vi "Measurement Logic.vi"(8 "error in":errorcluster, 9 "measurement configuration":T2 {"PAYLOAD" format="%x"; "TYPE" items=["CAN Data"=0, "CAN Remote"=1, "CAN Bus Error"=2, "CAN 2.0 Data"=8, "CAN FD Data"=16, "CAN FD+BRS Data"=24, "J1939 Data"=192, "Delay"=224, "Log Trigger"=225, "Start Trigger"=226]; "IDENTIFIER" format="%x"; "Baudrate" format="%x"; "FD Baudrate" format="%x"}, 10 "measure call context in":refnum<class "Measure Call Context.lvclass">) -> (0 "error out":errorcluster, 1 "measurement results":T1, 2 "measure call context out":refnum<class "Measure Call Context.lvclass">)   [LabVIEW 2025, in "CAN-LIN Frame Generator.lvclass"]
doc: "Contains the core logic for executing the measurement."
uses:
  CAN-LIN Frame Generator.lvclass
  <vilib>/Plug-In SDKs/Measurements/Measure Call Context/Measure Call Context.lvclass
  Measurement Configuration.ctl
  Measurement Results.ctl
  <vilib>/xnet/xnet.llb/XNET Frame CAN.ctl
  <vilib>/xnet/xnet.llb/XNET Frame Type CAN.ctl
  <vilib>/xnet/xnet.llb/XNET Create Session (Frame Output Stream).vi
  <extravilib>/ChannelInstances/Event Messenger-bool/Instantiate.vi
  CAN-LIN Frame Generator.lvclass/CAN-LIN Frame Generator.ctl
  <vilib>/xnet/xnet.llb/XNET Wait (Transmit Complete).vi
  <vilib>/xnet/xnet.llb/XNET Write (Frame CAN).vi
  <resource>/objmgr/xnet.rc
  session-management/xnetCAN/Session Management xnetCAN.lvlib
  <vilib>/Plug-In SDKs/Clients/Session Management V1/Session Reservation/Session Reservation.lvclass
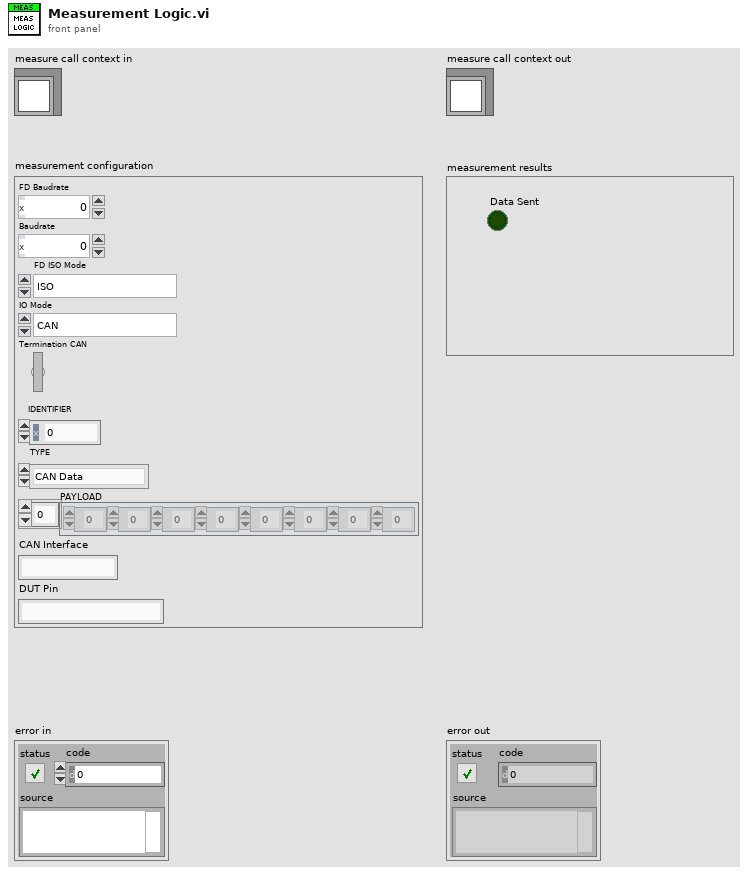
[diagram p1: front panel]
types:
  T1 = typedef "CAN-LIN Frame Generator.lvclass/Measurement Results.ctl" = cluster{"Data Sent":bool}
  T2 = typedef "CAN-LIN Frame Generator.lvclass/Measurement Configuration.ctl" = cluster{"FD Baudrate":u32, "Baudrate":u32, "FD ISO Mode":enum32{"ISO", "Legacy ISO", "Non-ISO"}, "IO Mode":enum32{"CAN", "CAN FD", "CAN FD + BRS"}, "Termination CAN":bool, "IDENTIFIER":u32, "TYPE":u32, "PAYLOAD":u32[], "CAN Interface":string, "DUT Pin":string}
  T3 = typedef "Session Management xnetCAN.lvlib/Connection with Session.ctl" = cluster{"connection":T4, "session":string}
  T4 = typedef "NI Session Management V1 Client.lvlib/Session Reservation.lvclass/Connection.ctl" = cluster{"pin or relay name":string, "site":i32, "instrument type id":string, "channel":string}
  T5 = typedef "XNET Frame CAN.ctl" = cluster{"timestamp":timestamp, "payload":u8[], "identifier":u32, "type":T6, "extended?":bool, "echo?":bool}
  T6 = typedef "XNET Frame Type CAN.ctl" = u8
  T7 = typedef "Event Messenger-bool.lvlib/))Channel.ctl" = refnum<queue>
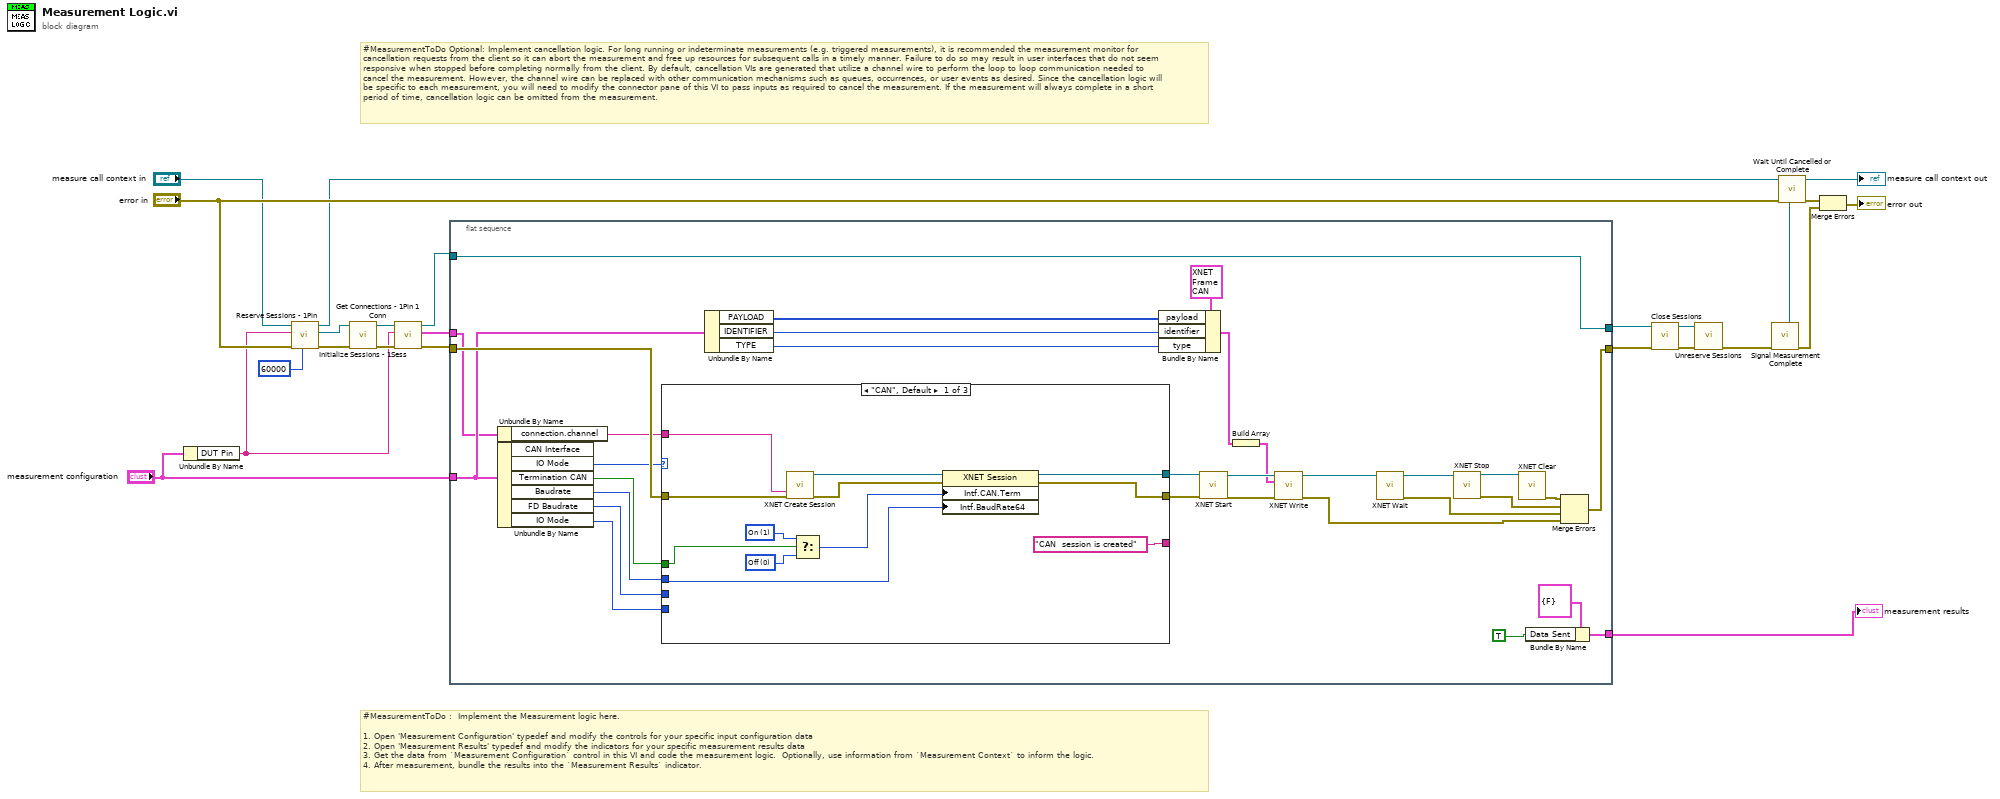
[diagram p0: block diagram]
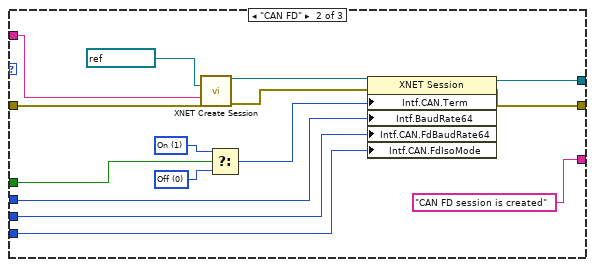
[diagram p2: hidden frame]
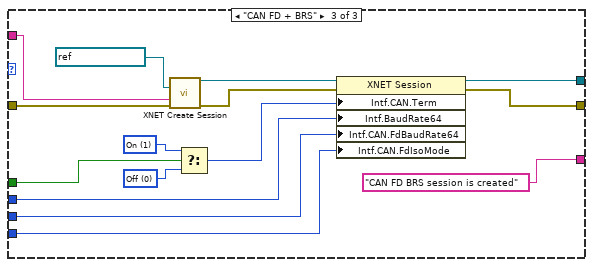
[diagram p3: hidden frame]
diagram:
  # "#MeasurementToDo Optional: Implement cancellation logic. For long running or indeterminate measurements (e.g. triggered measurements), it is recommended the measurement monitor for cancellation requests from the client so it can abort the measurement and free up resources for subsequent calls in a timely manner. Failure to do so may result in user interfaces that do not seem responsive when stopped before completing normally from the client. By default, cancellation VIs are generated that utilize a channel wire to perform the loop to loop communication needed to cancel the measurement. However, the channel wire can be replaced with other communication mechanisms such as queues, occurrences, or user events as desired. Since the cancellation logic will be specific to each measurement, you will need to modify the connector pane of this VI to pass inputs as required to cancel the measurement. If the measurement will always complete in a short period of time, cancellation logic can be omitted from the measurement."
  # "#MeasurementToDo :  Implement the Measurement logic here.\n\n1. Open 'Measurement Configuration' typedef and modify the controls for your specific input configuration data\n2. Open 'Measurement Results' typedef and modify the indicators for your specific measurement results data\n3. Get the data from `Measurement Configuration` control in this VI and code the measurement logic.  Optionally, use information from `Measurement Context` to inform the logic.\n4. After measurement, bundle the results into the `Measurement Results` indicator."
  n1 = Unbundle By Name("measurement configuration") -> ("DUT Pin"=w2:string)
  n2 = call <vilib>:"Reserve Sessions - 1Pin.vi"("timeout (ms)"=60000 ("timeout in milliseconds"), "error in"="error in", "pin or relay name"=w2, "measurement context in"="measure call context in") -> ("error out"=w13:errorcluster, "session reservation out"=w16:refnum<class "Session Reservation.lvclass">, "measurement context out"=w14:refnum<class "Measure Call Context.lvclass">)  [unwired: 5 in]
  n3 = call "Initialize Sessions - 1Sess.vi"("error in"=w13, "session reservation in"=w16) -> ("error out"=w5:errorcluster, "session reservation out"=w6:refnum<class "Session Reservation.lvclass">)  [unwired: 6 in, 2 out]
  n4 = call "Get Connections - 1Pin 1 Conn.vi"("error in"=w5, "pin or relay name"=w2, "session reservation in"=w6) -> ("error out"=w4:errorcluster, "connection"=w1:T3, "session reservation out"=w3:refnum<class "Session Reservation.lvclass">)  [unwired: 6 in]
  n5 = flat-sequence {
    tunnel: "measurement configuration" -> [w31]
    tunnel: w4 -> [w55]
    tunnel: [w33] -> w10
    tunnel: [w45] -> w19
    tunnel: [w27] -> w8
    tunnel: w3 -> [w27]
    tunnel: w1 -> [w26]
    frame #0 {
      n6 = Unbundle By Name(w26) -> ("connection.channel"=w25:string)
      n7 = Unbundle By Name(w31) -> ("IO Mode"=w43:enum32{"CAN", "CAN FD", "CAN FD + BRS"}, "Termination CAN"=w54:bool, "Baudrate"=w53:u32, "FD Baudrate"=w52:u32, "IO Mode"=w51:enum32{"CAN", "CAN FD", "CAN FD + BRS"})  [unwired: 1 out]
      n8 = case shown="\"CAN\", Default" w43 {
        tunnel: [w62 w72 w91] -> w50
        tunnel: w55 -> [w61 w76 w86]
        tunnel: [w60 w71 w85] -> w49
        tunnel: w54 -> [w59 w75 w90]
        tunnel: w53 -> [w58 w74 w89]
        tunnel: w52 -> [_ w70 w88]
        tunnel: w51 -> [_ w73 w87]
        tunnel: ["CAN  session is created" ("message") "CAN FD session is created" ("message") "CAN FD BRS session is created" ("message")] -> _
        tunnel: w25 -> [w56 w68 w83]
        frame "CAN", Default {
          w65 = u32 1 items=["Off", "On"] ("Interface:CAN:Termination")
          w64 = u32 0 items=["Off", "On"] ("Interface:CAN:Termination")
          n9 = call-poly <vilib>:"XNET Create Session.vi"("interface"=w56, "error in (no error)"=w61) -> ("session out"=w67:refnum<k21>, "error out"=w66:errorcluster)  [unwired: 12 in]
          n10 = Select(t=w65, s=w59, f=w64) -> (s? t:f=w63:u32)
          n11 = property class="XNET Session"(reference=w67, error in=w66, "Intf.CAN.Term"=w63, "Intf.BaudRate64"=w58) -> (reference out=w62:refnum<k21>, error out=w60:errorcluster)
        }
        frame "CAN FD" {
          w79 = u32 1 items=["Off", "On"] ("Interface:CAN:Termination")
          w78 = u32 0 items=["Off", "On"] ("Interface:CAN:Termination")
          n12 = call-poly <vilib>:"XNET Create Session.vi"("cluster (:memory:)"=refnum<k21> ":can_fd:", "interface"=w68, "error in (no error)"=w76) -> ("session out"=w81:refnum<k21>, "error out"=w80:errorcluster)  [unwired: 11 in]
          n13 = Select(t=w79, s=w75, f=w78) -> (s? t:f=w77:u32)
          n14 = property class="XNET Session"(reference=w81, error in=w80, "Intf.CAN.Term"=w77, "Intf.BaudRate64"=w74, "Intf.CAN.FdBaudRate64"=w70, "Intf.CAN.FdIsoMode"=w73) -> (reference out=w72:refnum<k21>, error out=w71:errorcluster)
        }
        frame "CAN FD + BRS" {
          w94 = u32 1 items=["Off", "On"] ("Interface:CAN:Termination")
          w93 = u32 0 items=["Off", "On"] ("Interface:CAN:Termination")
          n15 = call-poly <vilib>:"XNET Create Session.vi"("cluster (:memory:)"=refnum<k21> ":can_fd_brs:", "interface"=w83, "error in (no error)"=w86) -> ("session out"=w96:refnum<k21>, "error out"=w95:errorcluster)  [unwired: 11 in]
          n16 = Select(t=w94, s=w90, f=w93) -> (s? t:f=w92:u32)
          n17 = property class="XNET Session"(reference=w96, error in=w95, "Intf.CAN.Term"=w92, "Intf.BaudRate64"=w89, "Intf.CAN.FdBaudRate64"=w88, "Intf.CAN.FdIsoMode"=w87) -> (reference out=w91:refnum<k21>, error out=w85:errorcluster)
        }
      }
      n18 = Unbundle By Name(w31) -> ("PAYLOAD"=w30:u32[], "IDENTIFIER"=w29:u32, "TYPE"=w28:u32)
      n19 = Bundle By Name(cluster=T5 {"timestamp"=timestamp(0 s since 1904-01-01), "payload"=[1, 2, 3, 4, 5, 6, 7, 8], "identifier"=2, "type"=0, "extended?"=FALSE, "echo?"=FALSE} ("CAN frame"), "payload"=w30, "identifier"=w29, "type"=w28) -> (w41:T5)
      n20 = call <vilib>:"XNET Start.vi"("session in"=w50, "error in (no error)"=w49) -> ("session out"=w48:refnum<k21>, "error out"=w47:errorcluster)  [unwired: 12 in]
      n21 = Build Array(w41) -> (w40:T5[])
      n22 = call-poly <vilib>:"XNET Write.vi"("session in"=w48, "data"=w40, "error in (no error)"=w47) -> ("session out"=w39:refnum<k21>, "error out"=w32:errorcluster)  [unwired: 11 out]
      n23 = call-poly <vilib>:"XNET Wait.vi"("session in"=w39) -> ("session out"=w38:refnum<k21>, "error out"=w34:errorcluster)  [unwired: 13 in]
      n24 = call <vilib>:"XNET Stop.vi"("session in"=w38) -> ("session out"=w37:refnum<k21>, "error out"=w35:errorcluster)  [unwired: 13 in]
      n25 = call <vilib>:"XNET Clear.vi"("session in"=w37) -> ("error out"=w36:errorcluster)  [unwired: 14 in]
      n26 = Bundle By Name(cluster=T1 {"Data Sent"=FALSE} ("measurement results"), "Data Sent"=TRUE) -> (w45:T1)
      n27 = Merge Errors(w36, w35, w34, w32) -> (w33:errorcluster)
    }
  }
  n28 = call <vilib>:"Close Sessions.vi"("error in"=w10, "session reservation in"=w8) -> ("error out"=w12:errorcluster, "session reservation out"=w11:refnum<class "Session Reservation.lvclass">)  [unwired: 8 in]
  n29 = call <vilib>:"Unreserve Sessions.vi"("error in"=w12, "session reservation in"=w11) -> ("error out"=w9:errorcluster)  [unwired: 9 in]
  n30 = call "Signal Measurement Complete.vi"("error in (no error)"=w9) -> ("error out"=w22:errorcluster, "done channel"=w23:T7)  [unwired: 9 in]
  n31 = call "Wait Until Cancelled or Complete.vi"("done channel"=w23, "error in (no error)"="error in", "measure call context in"=w14) -> ("error out"=w21:errorcluster, "measure call context out"=→"measure call context out":refnum<class "Measure Call Context.lvclass">)  [unwired: 7 in]
  n32 = Merge Errors(w21, w22) -> (→"error out":errorcluster)
  "measurement results" <- w19
